vi "ZM-PC-init.vi"(8 "error in (no error)":errorcluster, 11 "ZM-PC-package in":refnum<class "ZM-PC-package.lvclass">) -> (0 "error out":errorcluster, 3 "ZM-PC-package out":refnum<class "ZM-PC-package.lvclass">)   [LabVIEW 2020, in "ZM-PC-packages.lvlib" / "ZM-PC-package.lvclass"]
doc: "Initialises a package (dynamic dispatch): writes the current time from Get Date/Time In Seconds through Write timestamp and the type Undefined through Write type. The destination is not touched. Each child overrides it with Call Parent followed by its own setType hook."
uses:
  ZM-PC-package.lvclass
  ZM-PC-package.lvclass/ZM-PC-package.ctl
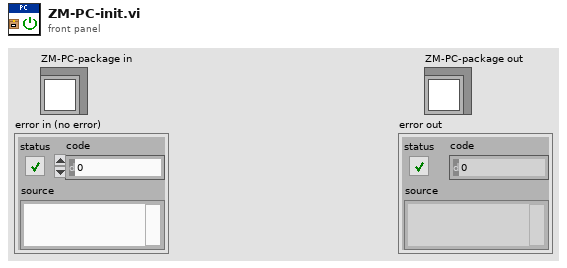
[diagram p1: front panel]
types:
  T1 = enum16{"Undefined", "TestPackage", "ErrorPackage"}
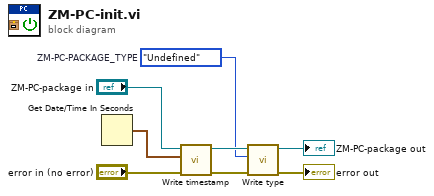
[diagram p0: block diagram]
diagram:
  w3 = T1."Undefined"  # ZM-PC-PACKAGE_TYPE
  n1 = Get Date/Time In Seconds() -> (seconds since 1Jan1904=w6:timestamp)
  n2 = call "Write timestamp.vi"("error in (no error)"="error in (no error)", "timestamp"=w6, "ZM-PC-package in"="ZM-PC-package in") -> ("error out"=w5:errorcluster, "ZM-PC-package out"=w4:refnum<class "ZM-PC-package.lvclass">)  [unwired: 7 in]
  n3 = call "Write type.vi"("error in (no error)"=w5, "ZM-PC-PACKAGE_TYPE"=w3, "ZM-PC-package in"=w4) -> ("error out"=→"error out":errorcluster, "ZM-PC-package out"=→"ZM-PC-package out":refnum<class "ZM-PC-package.lvclass">)  [unwired: 7 in]
